vi "Set Ann dx.vi"(8 "error in":errorcluster, 9 "Active Plot":u32, 10 "Points":cluster{"X":dbl, "Y":dbl}[](array[cluster]), 11 "XY Plot":refnum<vi>) -> (0 "error out":errorcluster, 3 "XY Plot out":refnum<vi>)   [LabVIEW 2025, in "XY Plotter.lvlib" / "XY Plotter.lvclass"]
uses:
  XY Plotter.lvclass
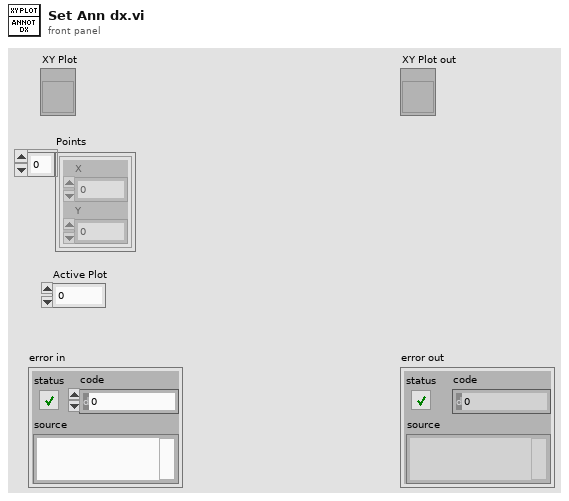
[diagram p1: front panel]
types:
  T1 = cluster{"Name":string, "Color":u32, "Style":u8, "Point Style":u8, "Name Visible":bool, "Allow Drag":bool, "Annotation Mode":u32, "Plot":i32, "Index":i32, "Position":cluster{"X":dbl, "Y":dbl}, "X Scale":u32, "Y Scale":u32, "Show Arrow":bool, "Lock Name":bool, "Plot Area":i32, "Label Offset":cluster{"X":dbl, "Y":dbl}}
  T2 = typedef "LVAnnotationListTypeDef.ctl" = cluster{"Name":string, "Color":u32, "Style":u8, "Point Style":u8, "Name Visible":bool, "Allow Drag":bool, "Annotation Mode":u32, "Plot":i32, "Index":i32, "Position":cluster{"X":dbl, "Y":dbl}, "X Scale":u32, "Y Scale":u32, "Show Arrow":bool, "Lock Name":bool, "Plot Area":i32, "Label Offset":cluster{"X":dbl, "Y":dbl}}[]
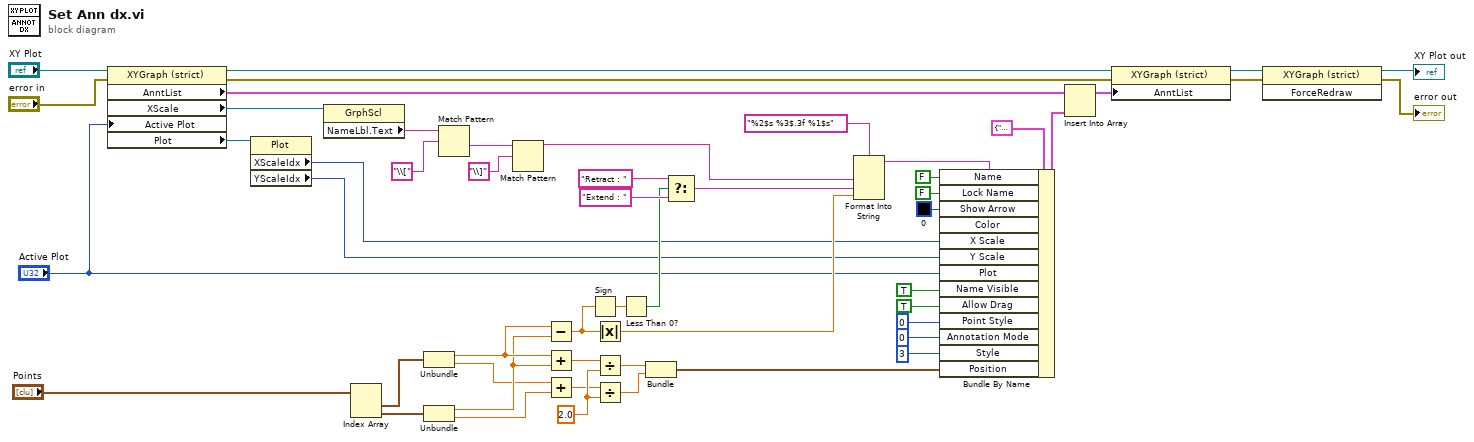
[diagram p0: block diagram]
diagram:
  w32 = 2.0 ("y")
  n1 = property class="XYGraph (strict)"(reference="XY Plot", error in="error in", "Active Plot"="Active Plot") -> (reference out=w45:refnum<vi>, error out=w44:errorcluster, "AnntList"=w46:T2, "XScale"=w41:refnum<vi>, "Plot"=w36:refnum<vi>)
  n2 = property class="Plot"(reference=w36) -> ("XScaleIdx"=w16:u32, "YScaleIdx"=w15:u32)  [unwired: 1 in, 2 out]
  n3 = property class="GrphScl"(reference=w41) -> ("NameLbl.Text"=w38:string)  [unwired: 1 in, 2 out]
  n4 = Index Array(array="Points") -> (element #1=w29:cluster{"X":dbl, "Y":dbl}, element #2=w30:cluster{"X":dbl, "Y":dbl})  [unwired: 2 in]
  n5 = Unbundle(w29) -> ("X"=w10:dbl, "Y"=w8:dbl)
  n6 = Unbundle(w30) -> ("X"=w9:dbl, "Y"=w7:dbl)
  n7 = Match Pattern(string=w38, regular expression="\\[") -> (after substring=w39:string)  [unwired: 1 in, 3 out]
  n8 = Match Pattern(string=w39, regular expression="\\]") -> (before substring=w25:string)  [unwired: 1 in, 3 out]
  n9 = Subtract(x=w10, y=w9) -> (x-y=w21:dbl)
  n10 = Add(x=w10, y=w9) -> (x+y=w33:dbl)
  n11 = Add(x=w8, y=w7) -> (x+y=w31:dbl)
  n12 = Sign(1:w21) -> (0:w22:dbl)
  n13 = Absolute Value(x=w21) -> (abs(x)=w18:dbl)
  n14 = Divide(x=w33, y=w32) -> (x/y=w34:dbl)
  n15 = Divide(x=w31, y=w32) -> (x/y=w35:dbl)
  n16 = Less Than 0?(x=w22) -> (x < 0?=w19:bool)
  n17 = Bundle(w34, w35) -> (w5:cluster{dbl, dbl})  [unwired: 1 in]
  n18 = Select(t="Retract : " ("format string"), s=w19, f="Extend : " ("format string")) -> (s? t:f=w17:string)
  n19 = Format Into String(format string="%2$s %3$.3f %1$s", w25, w17, w18) -> (resulting string=w11:string)  [unwired: 2 in, 1 out]
  n20 = Bundle By Name(cluster=T1 {"Name"="", "Color"=0, "Style"=0, "Point Style"=0, "Name Visible"=FALSE, "Allow Drag"=FALSE, "Annotation Mode"=0, "Plot"=0, "Index"=0, "Position"={"X"=0.0, "Y"=0.0}, "X Scale"=0, "Y Scale"=0, "Show Arrow"=FALSE, "Lock Name"=FALSE, "Plot Area"=0, "Label Offset"={"X"=0.0, "Y"=0.0}} ("new element/subarray"), "Name"=w11, "Lock Name"=FALSE, "Show Arrow"=FALSE, "Color"=u32 0, "X Scale"=w16, "Y Scale"=w15, "Plot"="Active Plot", "Name Visible"=TRUE, "Allow Drag"=TRUE, "Point Style"=u8 0, "Annotation Mode"=u32 0, "Style"=u8 3, "Position"=w5) -> (w47:T1)
  n21 = Insert Into Array(array=w46, new element=w47) -> (w52:T2)  [unwired: 1 in]
  n22 = property class="XYGraph (strict)"(reference=w45, error in=w44, "AnntList"=w52) -> (reference out=w2:refnum<vi>, error out=w50:errorcluster)
  n23 = invoke class="XYGraph (strict)" method="ForceRedraw"(reference=w2, error in=w50) -> (reference out=→"XY Plot out":refnum<vi>, error out=→"error out":errorcluster)  [unwired: 1 in, 1 out]
